vi "Open Reference to SubVI.vi"(8 "error in (no error)":errorcluster, 10 "SubVI Name":string, 11 "VI in":refnum<vi>) -> (0 "error out":errorcluster, 2 "SubVIs":refnum<vi>[](array[refnum]), 3 "VI out":refnum<vi>)   [LabVIEW 2020, in "Mock Class Generator.lvclass"]
uses:
  Mock Class Generator.lvclass
  <vilib>/Utility/traverseref.llb/TRef TravTarget.ctl
  <vilib>/Utility/traverseref.llb/VI Scripting - Traverse.lvlib
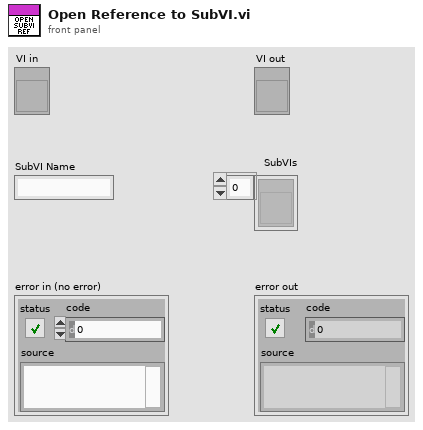
[diagram p1: front panel]
types:
  T1 = typedef "TRef TravTarget.ctl" = enum16{"FP", "BD", "Other"}
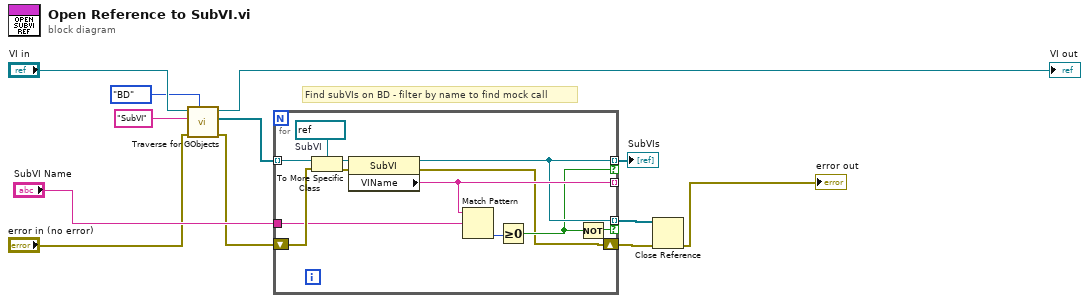
[diagram p0: block diagram]
diagram:
  # "Find subVIs on BD - filter by name to find mock call"
  n1 = call <vilib>:"Traverse for GObjects.vi"("Traverse Target"=TRef_TravTarget."BD", "error in (no error)"="error in (no error)", "Class Name"="SubVI", "VI Refnum"="VI in") -> ("error out"=w4:errorcluster, "References"=w3:refnum<vi>[], "dup VI Refnum"=→"VI out":refnum<vi>)  [unwired: 4 in, 1 out]
  n2 = for {
    tunnel: w3 -> [w24] mode=indexing
    tunnel: [w17] -> w1 mode=indexing if=w16
    tunnel: [w19] -> _ mode=indexing
    tunnel: [w17] -> w6 mode=indexing if=w15
    shift-right: [w14] -> w7
    shift-left: w4 -> [w20]
    tunnel: "SubVI Name" -> [w13]
    w22 = refnum<vi> refnum  # SubVI
    n3 = To More Specific Class(target class=w22, reference=w24, error in=w20) -> (specific class reference=w23:refnum<vi>, error out=w21:errorcluster)
    n4 = property class="SubVI"(reference=w23, error in=w21) -> (reference out=w17:refnum<vi>, error out=w14:errorcluster, "VIName"=w19:string)
    n5 = Match Pattern(string=w19, regular expression=w13) -> (offset past match=w18:i32)  [unwired: 1 in, 3 out]
    n6 = Greater Or Equal To 0?(x=w18) -> (x >= 0?=w16:bool)
    n7 = Not(x=w16) -> (.not. x?=w15:bool)
  }
  "SubVIs" <- w1
  n8 = Close Reference(reference=w6, error in (no error)=w7) -> (error out=→"error out":errorcluster)
